vi "LabApp - Setup Simulator.vi"(5 "cmd":enum16{"init", "get", "set"}(ring)=enum."get", 9 "control":dbl format="%.2f") -> (1 "param 2":dbl format="%.2f", 2 "param 1":dbl format="%.2f")   [LabVIEW 2021]
doc: "::: CalcExpress Toolkit :::\nCopyright (c) 2000-2026 Konstantin Shifershteyn. All rights reserved."
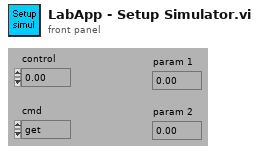
[diagram p1: front panel]
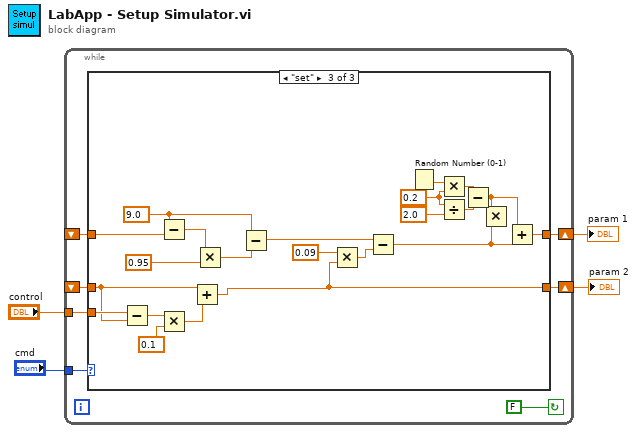
[diagram p0: block diagram]
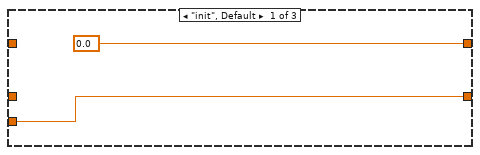
[diagram p2: hidden frame]
diagram:
  n1 = while {
    tunnel: "control" -> [w9]
    shift-left: _ -> [w6]
    shift-right: [w10] -> w1
    shift-left: _ -> [w7]
    shift-right: [w8] -> w2
    tunnel: "cmd" -> [w11]
    stop <- FALSE continue-if-true
    n2 = case shown="\"set\"" w11 {
      tunnel: [w13 w14 w30] -> w10
      tunnel: w9 -> [w13 _ w34]
      tunnel: [0.0 ("control") w15 w19] -> w8
      tunnel: w7 -> [_ w15 w29]
      tunnel: w6 -> [_ w14 w33]
      frame "init", Default {
      }
      frame "get" {
      }
      frame "set" {
        w23 = 0.2 ("y")
        w27 = 9.0 ("x")
        n3 = Subtract(x=w34, y=w33) -> (x-y=w37:dbl)
        n4 = Subtract(x=w27, y=w29) -> (x-y=w28:dbl)
        n5 = Multiply(x=w37, y=0.1) -> (x*y=w35:dbl)
        n6 = Add(x=w33, y=w35) -> (x+y=w30:dbl)
        n7 = Multiply(x=w28, y=0.95) -> (x*y=w26:dbl)
        n8 = Subtract(x=w27, y=w26) -> (x-y=w25:dbl)
        n9 = Multiply(x=0.09, y=w30) -> (x*y=w31:dbl)
        n10 = Subtract(x=w25, y=w31) -> (x-y=w18:dbl)
        n11 = Random Number (0-1)() -> (number: 0 to 1=w24:dbl)
        n12 = Multiply(x=w24, y=w23) -> (x*y=w21:dbl)
        n13 = Divide(x=w23, y=2.0) -> (x/y=w20:dbl)
        n14 = Subtract(x=w21, y=w20) -> (x-y=w17:dbl)
        n15 = Multiply(x=w17, y=w18) -> ()  [unwired: 1 out]
        n16 = Add(x=w17, y=w18) -> (x+y=w19:dbl)
      }
    }
  }
  "param 1" <- w2
  "param 2" <- w1
